vi "Unary routeguide_RouteGuide_GetFeature.vi"(8 "error in":errorcluster, 10 "Request Data":T2, 11 "gRPC ID":T3) -> (0 "error out":errorcluster, 2 "Response Data":T1, 3 "gRPC ID out":T3)   [LabVIEW 2019, in "route_guide_client.lvlib"]
uses:
  route_guide_client.lvlib
  RPC Messages/routeguide_Point.ctl
  RPC Messages/routeguide_Feature.ctl
  e41a4c49-c94f-4bdb-bf87-ae25b439dcbc.vi
  <vilib>/gRPC/LabVIEW gRPC Library/Shared/grpcId.ctl
  <vilib>/gRPC/LabVIEW gRPC Library/grpc-lvsupport-release.lvlib
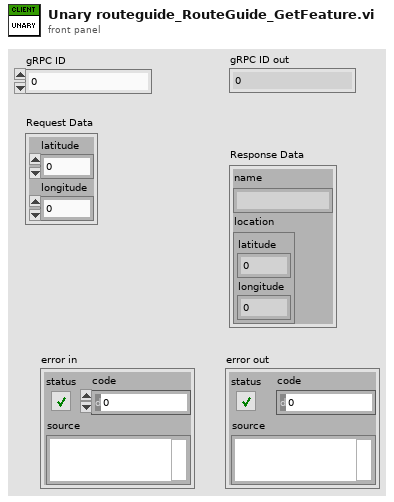
[diagram p1: front panel]
types:
  T1 = typedef "route_guide_client.lvlib/routeguide_Feature.ctl" = cluster{"name":string, "location":T2}
  T2 = typedef "route_guide_client.lvlib/routeguide_Point.ctl" = cluster{"latitude":i32, "longitude":i32}
  T3 = typedef "grpc-lvsupport-release.lvlib/grpcId.ctl" = u64
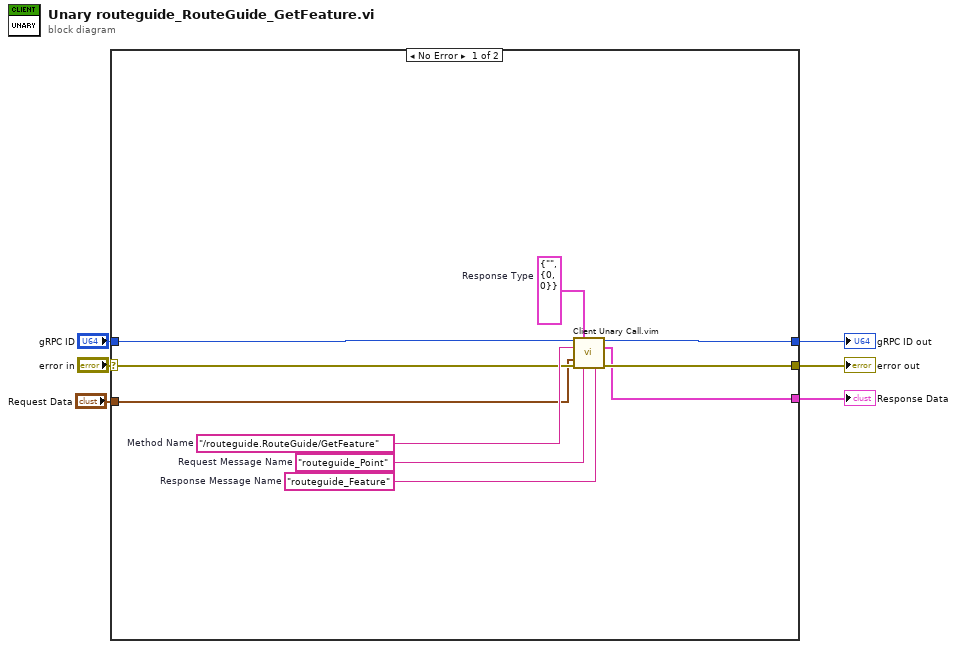
[diagram p0: block diagram]
diagram:
  n1 = case shown="No Error" "error in" {
    selector: "error in" -> [w12 w17]
    tunnel: [w11 w17] -> w5
    tunnel: "gRPC ID" -> [w10 w18]
    tunnel: [w9 w18] -> w3
    tunnel: "Request Data" -> [w8 _]
    tunnel: [w7 _] -> w1
    frame No Error {
      w13 = "routeguide_Feature"  # Response Message Name
      w14 = "routeguide_Point"  # Request Message Name
      w15 = T1 {"name"="", "location"={"latitude"=0, "longitude"=0}}  # Response Type
      w16 = "/routeguide.RouteGuide/GetFeature"  # Method Name
      n2 = call "Client Unary Call.vim"("ClientID in"=w10, "Response Type"=w15, "Method Name"=w16, "Request Data"=w8, "error in"=w12, "Request Message Name"=w14, "Response Message Name"=w13) -> ("ClientID out"=w9:u64, "Response Data"=w7:T1, "error out"=w11:errorcluster)  [unwired: 6 in]
    }
    frame Error {
    }
  }
  "error out" <- w5
  "gRPC ID out" <- w3
  "Response Data" <- w1
